vi "Untitled 5.vi"(11 "N":i32) -> (0 "FAC":i32)   [LabVIEW 2012]
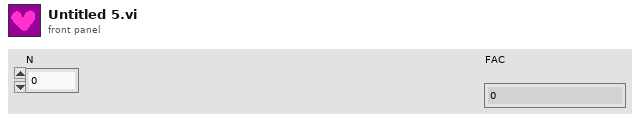
[diagram p1: front panel]
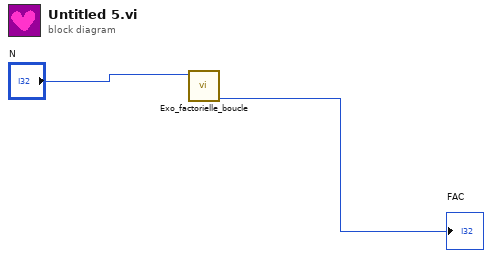
[diagram p0: block diagram]
diagram:
  n1 = call "Exo_factorielle_boucle.vi"("N"="N") -> ("resultat du facto"=→"FAC":i32)  [unwired: 10 in]
